vi "SendPacket.vi"(8 "error in":errorcluster, 10 "Ethernet Port Opened ?":bool, 11 "Packet Array":string[](array[string])) -> (0 "error out":errorcluster, 3 "Time per plane":u32)   [LabVIEW 2020]
panel:
  out "Ethernet Port Open":bool
  out "FOR Loop":i32
  out "Read Array":string[](array[string])
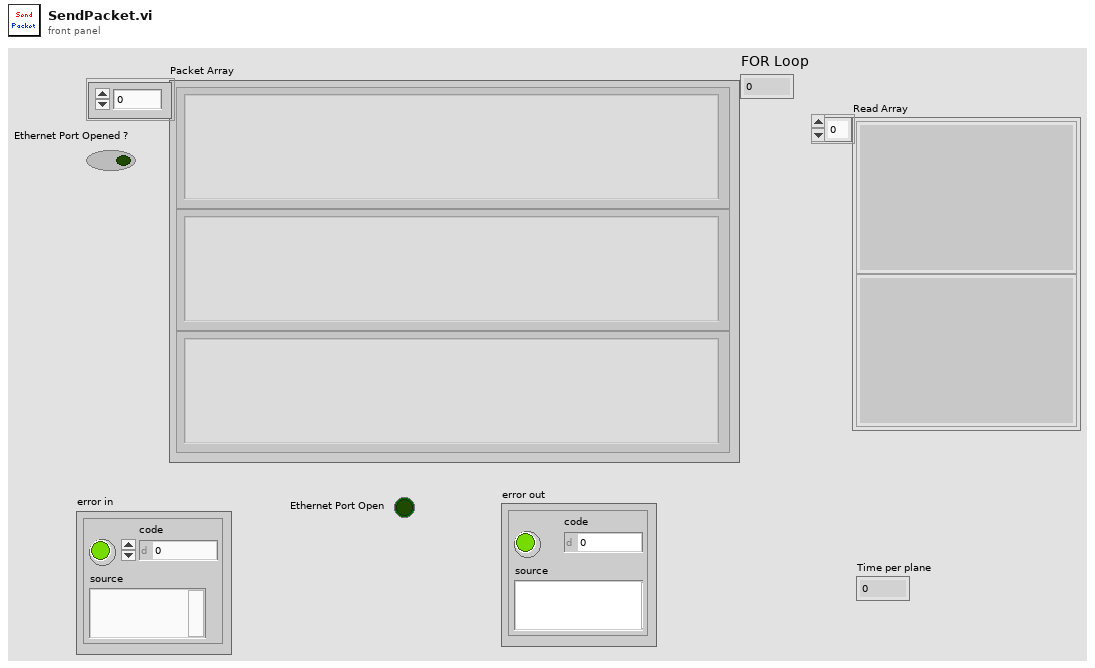
[diagram p1: front panel]
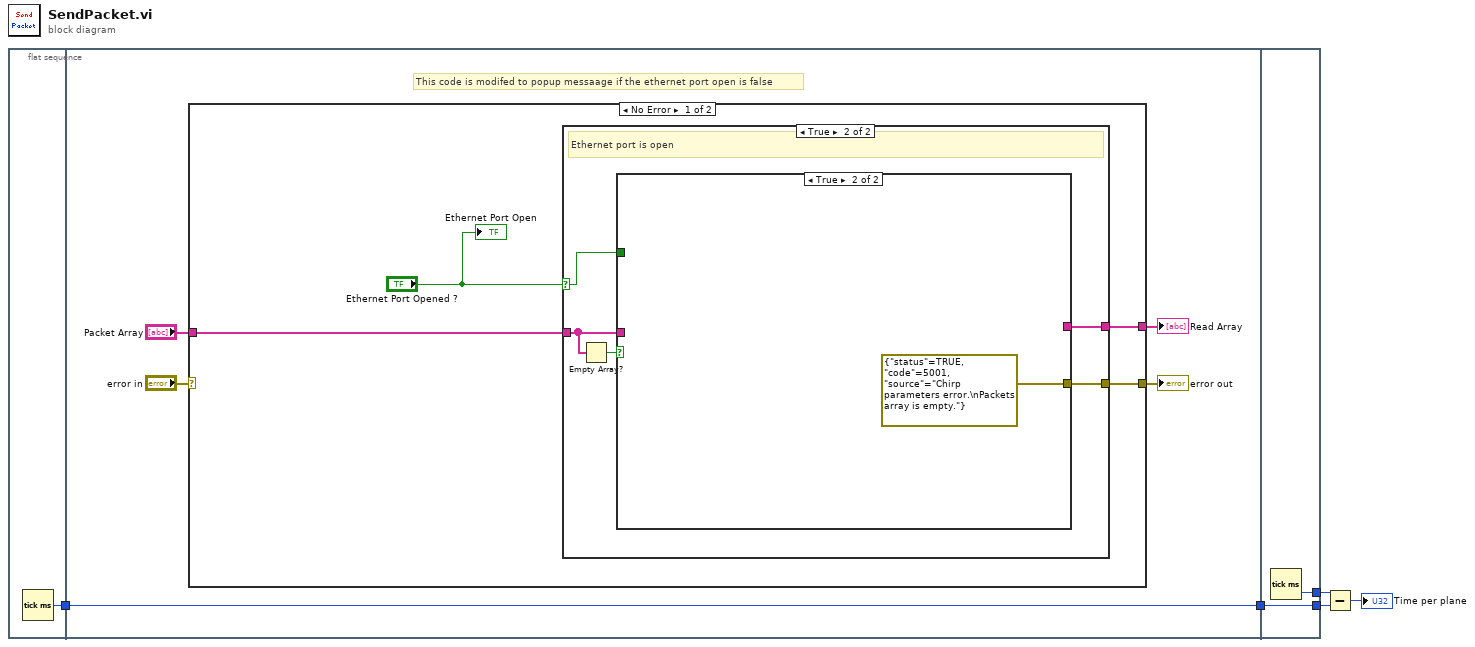
[diagram p0: block diagram]
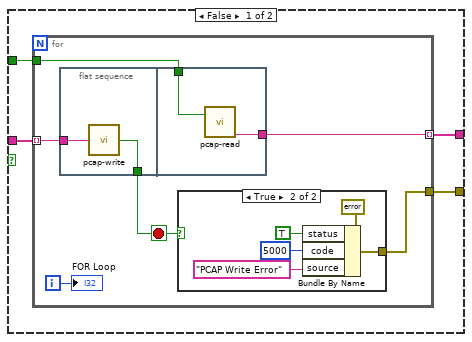
[diagram p3: hidden frame]
diagram:
  n1 = flat-sequence {
    tunnel: [w6] -> w4
    tunnel: w4 -> [w7]
    tunnel: [w7] -> w3
    tunnel: [w43] -> w5
    tunnel: w3 -> [w42]
    tunnel: [w42] -> w2
    frame #0 {
      n2 = Tick Count (ms)() -> (millisecond timer value=w6:u32)
    }
    frame #1 {
      # "This code is modifed to popup messaage if the ethernet port open is false"
      n3 = case shown="No Error" "error in" {
        selector: "error in" -> [_ w41]
        tunnel: "Packet Array" -> [w14 _]
        tunnel: [w15 w41] -> w10
        tunnel: [w13 _] -> w8
        frame No Error {
          n4 = case shown="True" "Ethernet Port Opened ?" {
            selector: "Ethernet Port Opened ?" -> [_ w16]
            tunnel: [_ w19] -> w15
            tunnel: w14 -> [_ w18]
            tunnel: [_ w20] -> w13
            frame False {
              # "Ethernet port is closed"
            }
            frame True {
              # "Ethernet port is open"
              n5 = Empty Array?(array=w18) -> (empty?=w17:bool)
              n6 = case shown="True" w17 {
                tunnel: w18 -> [w24 _]
                tunnel: [w23 _] -> w20
                tunnel: [w22 errorcluster {"status"=TRUE, "code"=5001, "source"="Chirp parameters error.\nPackets array is empty."} ("error out")] -> w19
                tunnel: w16 -> [w21 _]
                frame False {
                  n7 = for {
                    tunnel: w24 -> [w30] mode=indexing
                    tunnel: [w29] -> w23 mode=indexing
                    tunnel: [w27] -> w22
                    tunnel: w21 -> [w25]
                    i -> [w28]
                    stop <- w26 stop-if-true
                    n8 = flat-sequence {
                      tunnel: [w37] -> w26
                      tunnel: w30 -> [w36]
                      tunnel: [w39] -> w29
                      tunnel: w25 -> [w38]
                      frame #0 {
                        n9 = call "pcap-write.vi"("Data to Write"=w36) -> ("Write Error"=w37:bool)
                      }
                      frame #1 {
                        n10 = call "pcap-read.vi"("Opened"=w38) -> ("Packet Data:"=w39:string)  [unwired: 6 out]
                      }
                    }
                    n11 = case shown="True" w26 {
                      tunnel: [_ w33] -> w27
                      frame False {
                      }
                      frame True {
                        n12 = Bundle By Name(cluster=errorcluster {"status"=FALSE, "code"=0, "source"=""} ("error out"), "status"=TRUE, "code"=5000, "source"="PCAP Write Error") -> (w33:errorcluster)
                      }
                    }
                    "FOR Loop" <- w28
                  }
                }
                frame True {
                }
              }
            }
          }
          "Ethernet Port Open" <- "Ethernet Port Opened ?"
        }
        frame Error {
        }
      }
      "error out" <- w10
      "Read Array" <- w8
    }
    frame #2 {
      n13 = Tick Count (ms)() -> (millisecond timer value=w43:u32)
    }
  }
  n14 = Subtract(x=w5, y=w2) -> (x-y=→"Time per plane":u32)
